vi "Doubler.vi"(10 "Input":dbl) -> (2 "output":dbl)   [LabVIEW 2026]
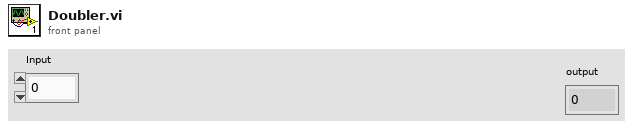
[diagram p1: front panel]
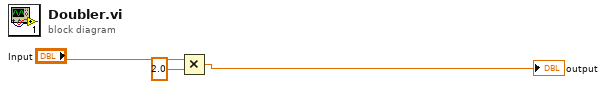
[diagram p0: block diagram]
diagram:
  n1 = Multiply(x="Input", y=2.0) -> (x*y=→"output":dbl)
